vi "G4SubTemplate_Singleton_6x8x6_CleanUp.vi"(5 "Error In":errorcluster) -> (19 "Error Out":errorcluster)   [LabVIEW 2020, in "G4SubTemplate_Singleton_6x8x6.lvclass"]
uses:
  G4SubTemplate_Singleton_6x8x6.lvclass
  G4BaseTemplate_Singleton_6x8x6/G4BaseTemplate_Singleton_6x8x6.lvclass
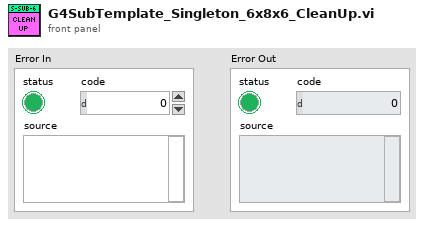
[diagram p1: front panel]
types:
  T1 = typedef "G4SubTemplate_Singleton_6x8x6.lvclass/ObjectAttributes.ctl" = cluster{"Attribute1":dbl}
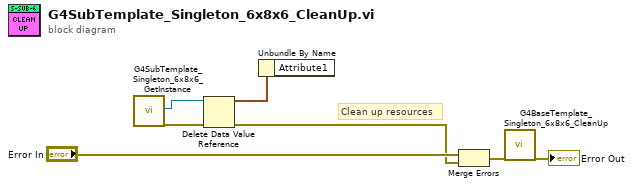
[diagram p0: block diagram]
diagram:
  # "Clean up resources"
  n1 = call "G4SubTemplate_Singleton_6x8x6_GetInstance.vi"() -> ("DVRRefOut"=w3:refnum<data-value>, "Error Out"=w1:errorcluster)  [unwired: 15 in, 3 out]
  n2 = Delete Data Value Reference(data value reference=w3, error in=w1) -> (data value=w2:T1, error out=w4:errorcluster)
  n3 = Unbundle By Name(w2) -> ()  [unwired: 1 out]
  n4 = Merge Errors("Error In", w4) -> (w7:errorcluster)
  n5 = call "G4BaseTemplate_Singleton_6x8x6_CleanUp.vi"("Error In"=w7) -> ("Error Out"=→"Error Out":errorcluster)  [unwired: 18 in]
